vi "VIH HelpGen - Open VI Reference.vi"(6 "Enable Conpane Image Check (T)":bool=TRUE, 8 "error in":errorcluster, 10 "Force use wrapper (F)":bool, 11 "VI Path":path) -> (0 "error out":errorcluster, 1 "Conpane Image":T1, 2 "Original VI Name":string, 3 "VI Reference":refnum<vi>)   [LabVIEW 2014]
doc: "::: VI Helpeks :::\nCopyright (c) 2000-2026 Konstantin Shifershteyn. All rights reserved."
uses:
  <vilib>/picture/picture.llb/imagedata.ctl
panel:
  # "VI Helpeks\nCopyright (c) 2012-2026 Konstantin Shifershteyn"
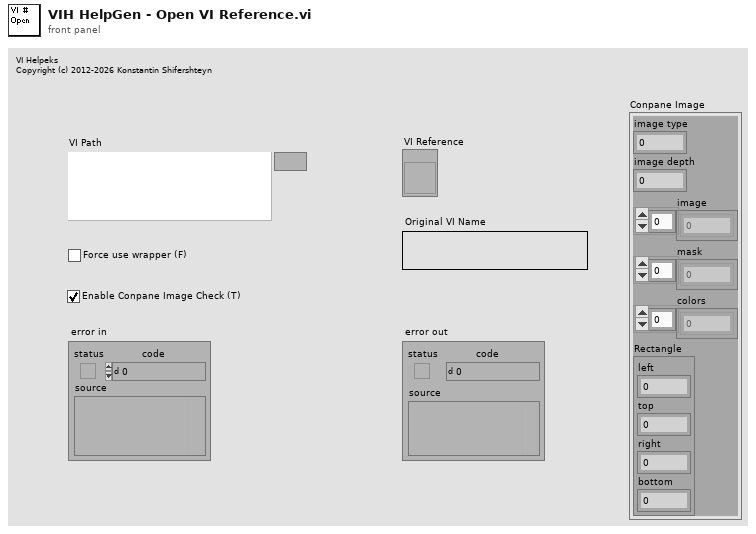
[diagram p1: front panel]
types:
  T1 = typedef "imagedata.ctl" = cluster{"image type":i32, "image depth":i32, "image":u8[], "mask":u8[], "colors":u32[], "Rectangle":cluster{"left":i16, "top":i16, "right":i16, "bottom":i16}}
  T2 = enum32{"Bad", "Idle", "Run top level", "Running"}
  T3 = cluster{"ShowQuickTips":bool, "NextQuickTip":i32, "FastLoadVI":bool, "EditPrgs ":cluster{"FileExtension":string, "CustProgram":path, "UseCustPrg":bool}[]}
  T4 = enum32{"invalid lock state", "Not Locked", "Locked (No Password)", "Password-protected"}
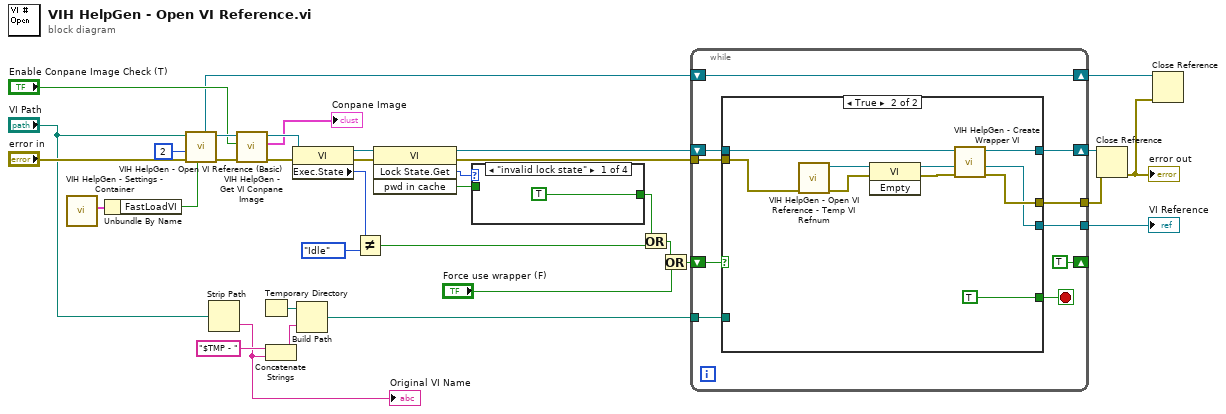
[diagram p0: block diagram]
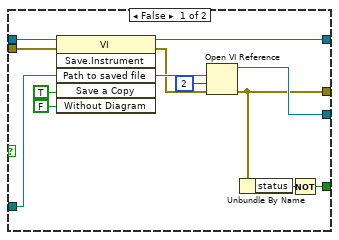
[diagram p2: hidden frame]
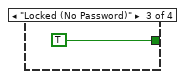
[diagram p4: hidden frame]
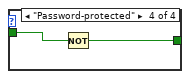
[diagram p5: hidden frame]
diagram:
  n1 = call "VIH HelpGen - Settings - Container.vi"() -> ("Settings out"=w5:T3)  [unwired: 10 in, 1 out]
  n2 = Unbundle By Name(w5) -> ("FastLoadVI"=w4:bool)
  n3 = call "VIH HelpGen - Open VI Reference (Basic).vi"("Without Refees (F)"=w4, "error in"="error in", "options"=2, "VI Path"="VI Path") -> ("error out"=w13:errorcluster, "VI Reference"=w12:refnum<vi>, "Tmp App Refnum"=w3:refnum<vi>)  [unwired: 5 in]
  n4 = Strip Path(path="VI Path") -> (name=w15:string)  [unwired: 1 out]
  "Original VI Name" <- w15
  n5 = call "VIH HelpGen - Get VI Conpane Image.vi"("error in"=w13, "Enable Check (T)"="Enable Conpane Image Check (T)", "VI Reference"=w12) -> ("error out"=w11:errorcluster, "Conpane Image"=→"Conpane Image":T1, "dup VI Reference"=w10:refnum<vi>)  [unwired: 6 in]
  n6 = Temporary Directory() -> (w34:path)
  n7 = Concatenate Strings("$TMP - ", w15) -> (w33:string)
  n8 = property class="VI"(reference=w10, error in=w11) -> (reference out=w22:refnum<vi>, error out=w21:errorcluster, "Exec.State"=w20:T2)
  n9 = Build Path(base path=w34, name or relative path=w33) -> (appended path=w31:path)
  n10 = Not Equal?(x=w20, y=T2."Idle" ("Execution:State")) -> (x != y?=w18:bool)
  n11 = invoke class="VI" method="Lock State.Get"(reference=w22, error in=w21) -> (reference out=w23:refnum<vi>, error out=w28:errorcluster, "Get Lock State"=w27:T4, "pwd in cache"=w26:bool)  [unwired: 2 in]
  n12 = case shown="\"invalid lock state\"" w27 {
    tunnel: w26 -> [_ _ _ w39]
    tunnel: [TRUE _ TRUE w38] -> w17
    frame "invalid lock state" {
    }
    frame "Not Locked" {
    }
    frame "Locked (No Password)" {
    }
    frame "Password-protected" {
      n13 = Not(x=w39) -> (.not. x?=w38:bool)
    }
  }
  n14 = Or(x=w17, y=w18) -> (x .or. y?=w16:bool)
  n15 = Or(x=w16, y="Force use wrapper (F)") -> (x .or. y?=w24:bool)
  n16 = while {
    tunnel: w31 -> [w48]
    tunnel: [w47] -> w14
    tunnel: [w46] -> w29
    tunnel: w28 -> [w45]
    shift-right: [w49] -> w32
    shift-left: w23 -> [w43]
    shift-right: [TRUE] -> _
    shift-left: w24 -> [w44]
    shift-right: [w40] -> w2
    shift-left: w3 -> [w40]
    stop <- w42 stop-if-true
    n17 = case shown="True" w44 {
      tunnel: [w59 w70] -> w49
      tunnel: w48 -> [w58 _]
      tunnel: [w57 w68] -> w47
      tunnel: [w53 w69] -> w46
      tunnel: w45 -> [w55 w64]
      tunnel: w43 -> [w54 w71]
      tunnel: [w51 TRUE] -> w42
      frame False {
        n18 = invoke class="VI" method="Save.Instrument"(reference=w54, error in=w55, "Path to saved file"=w58, "Save a Copy"=TRUE, "Without Diagram"=FALSE) -> (reference out=w59:refnum<vi>, error out=w56:errorcluster)  [unwired: 1 in, 4 out]
        n19 = Open VI Reference(vi path=w58, options=2, error in (no error)=w56) -> (vi reference=w57:refnum<vi>, error out=w53:errorcluster)  [unwired: 3 in]
        n20 = Unbundle By Name(w53) -> ("status"=w52:bool)
        n21 = Not(x=w52) -> (.not. x?=w51:bool)
      }
      frame True {
        n22 = call "VIH HelpGen - Open VI Reference - Temp VI Refnum.vi"("error in"=w64) -> ("error out"=w63:errorcluster, "VI Refnum"=w67:refnum<vi>)  [unwired: 9 in]
        n23 = invoke class="VI" method="Empty"(reference=w67, error in=w63) -> (reference out=w66:refnum<vi>, error out=w62:errorcluster)  [unwired: 1 in, 1 out]
        n24 = call "VIH HelpGen - Create Wrapper VI.vi"("error in"=w62, "Wrapper VI Refnum (opt)"=w66, "Original VI Refnum"=w71) -> ("error out"=w69:errorcluster, "Wrapper VI Refnum"=w68:refnum<vi>, "dup Original VI Refnum"=w70:refnum<vi>)  [unwired: 6 in]
      }
    }
  }
  "VI Reference" <- w14
  n25 = Close Reference(reference=w32, error in (no error)=w29) -> (error out=w1:errorcluster)
  "error out" <- w1
  n26 = Close Reference(reference=w2, error in (no error)=w1) -> ()  [unwired: 1 out]
